vi "Get Tunnel Ref by Name (Structure).vi"(8 "error IO":errorcluster, 9 "Input Tunnel (F)/Output Tunnel (T)":bool, 10 "Terminal Wire":string, 11 "Case Refnum In":refnum<vi>) -> (0 "error out":errorcluster, 2 "Desired Tunnel Reference":refnum<vi>, 3 "Case Refnum Out":refnum<vi>)   [LabVIEW 2012, in "Scripting Tools.lvlib"]
uses:
  Scripting Tools.lvlib
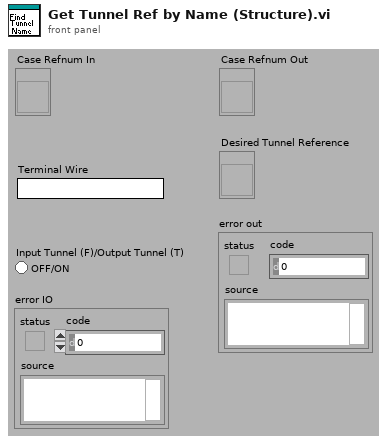
[diagram p1: front panel]
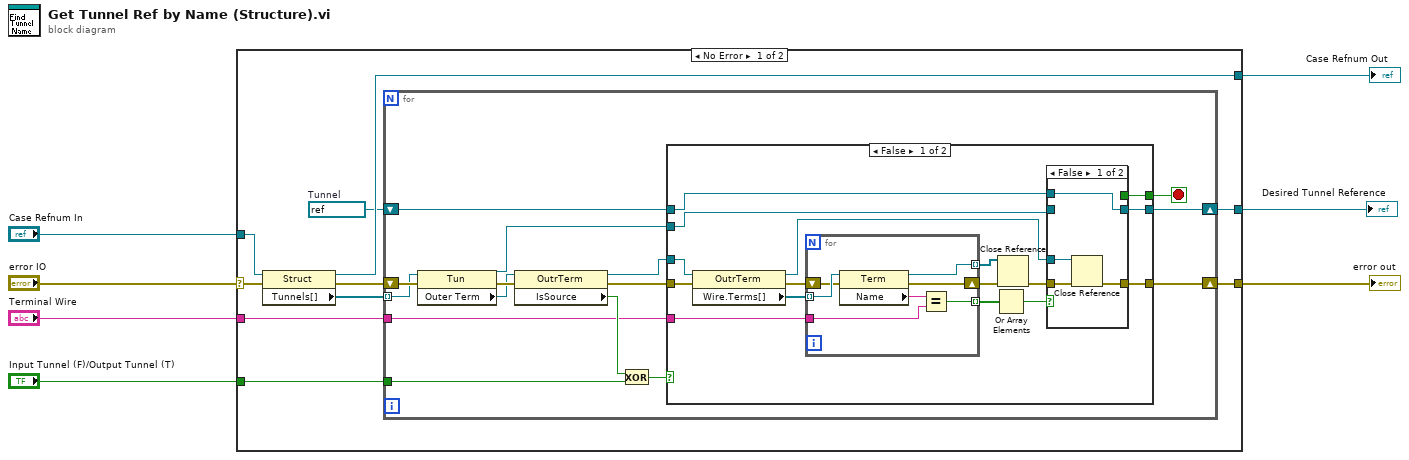
[diagram p0: block diagram]
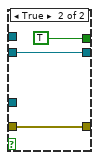
[diagram p2: hidden frame]
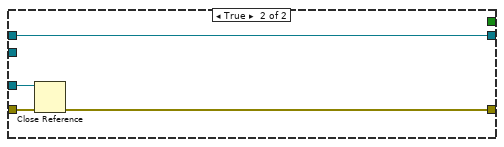
[diagram p3: hidden frame]
diagram:
  n1 = case shown="No Error" "error IO" {
    selector: "error IO" -> [w8 w67]
    tunnel: [w17 _] -> w7
    tunnel: [w16 w67] -> w6
    tunnel: "Input Tunnel (F)/Output Tunnel (T)" -> [w15 _]
    tunnel: "Terminal Wire" -> [w14 _]
    tunnel: [w13 _] -> w2
    tunnel: "Case Refnum In" -> [w9 _]
    frame No Error {
      w12 = refnum<vi> refnum  # Tunnel
      n2 = property class="Struct"(reference=w9, error in=w8) -> (reference out=w13:refnum<vi>, error out=w10:errorcluster, "Tunnels[]"=w11:refnum<vi>[])
      n3 = for {
        shift-right: [w22] -> w16
        shift-left: w10 -> [w32]
        tunnel: w11 -> [w31] mode=indexing
        shift-right: [w26] -> w17
        shift-left: w12 -> [w23]
        tunnel: w14 -> [w21]
        tunnel: w15 -> [w19]
        stop <- w18 stop-if-true
        n4 = property class="Tun"(reference=w31, error in=w32) -> (reference out=w24:refnum<vi>, error out=w30:errorcluster, "Outer Term"=w25:refnum<vi>)
        n5 = property class="OutrTerm"(reference=w25, error in=w30) -> (reference out=w28:refnum<vi>, error out=w27:errorcluster, "IsSource"=w29:bool)
        n6 = Exclusive Or(1:w19, 2:w29) -> (0:w20:bool)
        n7 = case shown="False" w20 {
          tunnel: w28 -> [w47 w65]
          tunnel: w27 -> [w48 w64]
          tunnel: [w45 w66] -> w26
          tunnel: w24 -> [w44 _]
          tunnel: w23 -> [w43 w66]
          tunnel: [w42 w63] -> w22
          tunnel: w21 -> [w39 _]
          tunnel: [w41 _] -> w18
          frame False {
            n8 = property class="OutrTerm"(reference=w47, error in=w48) -> (reference out=w46:refnum<vi>, error out=w35:errorcluster, "Wire.Terms[]"=w40:refnum<vi>[])
            n9 = for {
              tunnel: w40 -> [w55] mode=indexing
              tunnel: w39 -> [w53]
              tunnel: [w52] -> w38 mode=indexing
              tunnel: [w51] -> w36 mode=indexing
              shift-right: [w49] -> w34
              shift-left: w35 -> [w50]
              n10 = property class="Term"(reference=w55, error in=w50) -> (reference out=w51:refnum<vi>, error out=w49:errorcluster, "Name"=w54:string)
              n11 = Equal?(x=w54, y=w53) -> (x = y?=w52:bool)
            }
            n12 = Or Array Elements(Boolean array=w38) -> (logical OR=w37:bool)
            n13 = Close Reference(reference=w36, error in (no error)=w34) -> (error out=w33:errorcluster)
            n14 = case shown="False" w37 {
              tunnel: w46 -> [w58 _]
              tunnel: [w59 w62] -> w45
              tunnel: w44 -> [_ w62]
              tunnel: w43 -> [w59 _]
              tunnel: [w57 w60] -> w42
              tunnel: [_ TRUE] -> w41
              tunnel: w33 -> [w56 w60]
              frame False {
                n15 = Close Reference(reference=w58, error in (no error)=w56) -> (error out=w57:errorcluster)
              }
              frame True {
              }
            }
          }
          frame True {
            n16 = Close Reference(reference=w65, error in (no error)=w64) -> (error out=w63:errorcluster)
          }
        }
      }
    }
    frame Error {
    }
  }
  "Desired Tunnel Reference" <- w7
  "error out" <- w6
  "Case Refnum Out" <- w2
